vi "FuncVI_Sub - Script - Path argument to script path.vi"(6 "Allow Dialog (T)":bool=TRUE, 7 "CSE RefNum":T1, 8 "error in":errorcluster, 9 "prompt":string, 11 "arg: path":string) -> (0 "error out":errorcluster, 3 "script path":path)   [LabVIEW 2021]
doc: "::: CalcExpress Toolkit :::\nCopyright (c) 2000-2026 Konstantin Shifershteyn. All rights reserved."
uses:
  cse.llb/CSE Instance RefNum.ctl
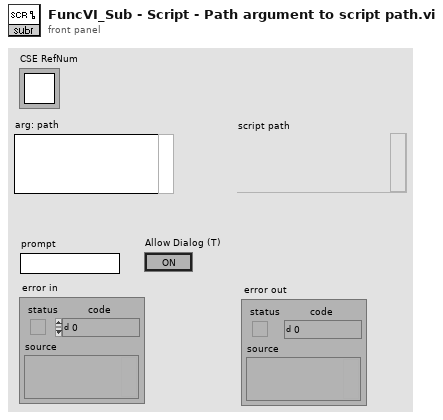
[diagram p1: front panel]
types:
  T1 = typedef "CSE Instance RefNum.ctl" = refnum<k1>
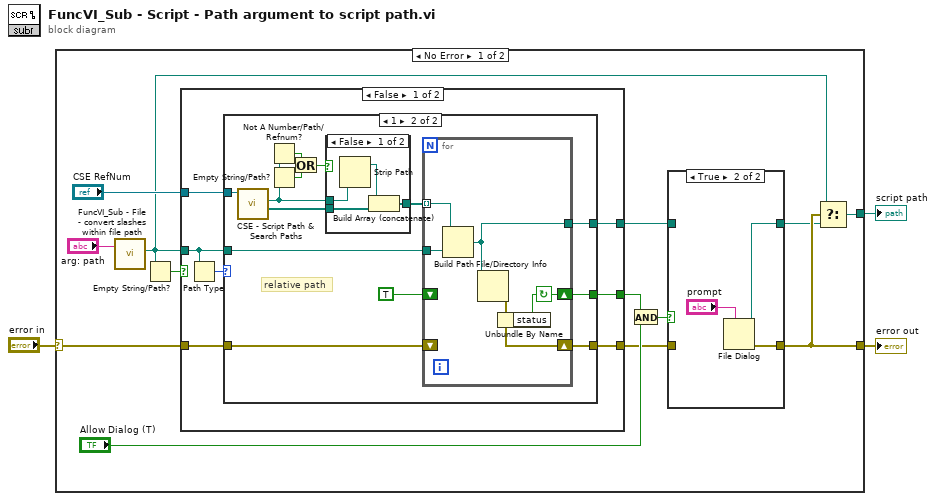
[diagram p0: block diagram]
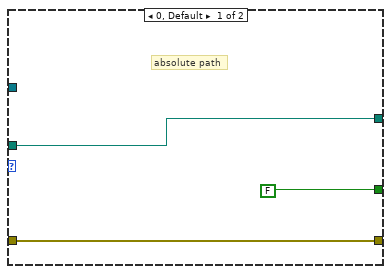
[diagram p3: hidden frame]
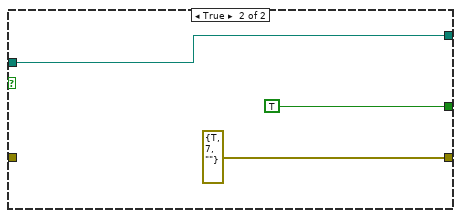
[diagram p5: hidden frame]
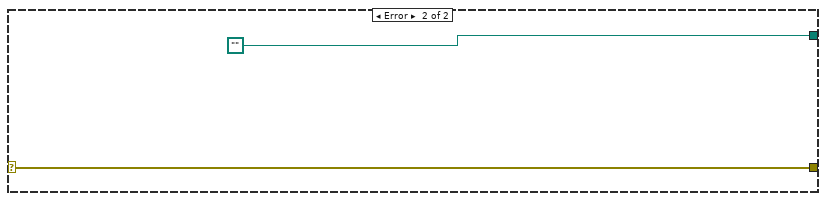
[diagram p6: hidden frame]
diagram:
  n1 = case shown="No Error" "error in" {
    selector: "error in" -> [w15 w58]
    tunnel: [w12 path ""] -> w3
    tunnel: [w6 w58] -> w2
    frame No Error {
      n2 = call "FuncVI_Sub - File - convert slashes within file path.vi"("str: path"="arg: path") -> ("path out"=w11:path)  [unwired: 3 in, 1 out]
      n3 = Empty String/Path?(string/path=w11) -> (empty?=w16:bool)
      n4 = case shown="False" w16 {
        tunnel: [w28 w55] -> w5
        tunnel: w11 -> [w23 w55]
        tunnel: w15 -> [w24 _]
        tunnel: [w25 errorcluster {"status"=TRUE, "code"=7, "source"=""} ("error out")] -> w7
        tunnel: "CSE RefNum" -> [w26 _]
        tunnel: [w22 TRUE] -> w10
        frame False {
          n5 = Path Type(1:w23) -> (0:w27:i16)
          n6 = case shown="1" w27 {
            tunnel: w23 -> [w30 w43]
            tunnel: [w30 w41] -> w28
            tunnel: w26 -> [_ w44]
            tunnel: [w31 w42] -> w25
            tunnel: w24 -> [w31 w33]
            tunnel: [FALSE w34] -> w22
            frame 0, Default {
              # "absolute path"
            }
            frame 1 {
              # "relative path"
              n7 = call "CSE - Script Path & Search Paths.vi"("CSE RefNum"=w44) -> ("search paths out"=w40:path[], "script file path out"=w37:path)  [unwired: 7 in, 2 out]
              n8 = Not A Number/Path/Refnum?(number/path/refnum=w37) -> (NaN/Path/Refnum?=w35:bool)
              n9 = Empty String/Path?(string/path=w37) -> (empty?=w36:bool)
              n10 = Or(x=w35, y=w36) -> (x .or. y?=w38:bool)
              n11 = case shown="False" w38 {
                tunnel: w40 -> [w53 w54]
                tunnel: [w52 w54] -> w39
                tunnel: w37 -> [w51 _]
                frame False {
                  n12 = Strip Path(path=w51) -> (stripped path=w50:path)  [unwired: 1 out]
                  n13 = Build Array (concatenate)(w50, w53) -> (w52:path[])
                }
                frame True {
                }
              }
              n14 = for {
                tunnel: w43 -> [w49]
                tunnel: w39 -> [w46] mode=indexing
                tunnel: [w47] -> w41
                shift-right: [w48] -> w42
                shift-left: w33 -> [_]
                shift-right: [w45] -> w34
                shift-left: TRUE -> [_]
                stop <- w45 continue-if-true
                n15 = Build Path(base path=w46, name or relative path=w49) -> (appended path=w47:path)
                n16 = File/Directory Info(path=w47) -> (error out=w48:errorcluster)  [unwired: 1 in, 6 out]
                n17 = Unbundle By Name(w48) -> ("status"=w45:bool)
              }
            }
          }
        }
        frame True {
        }
      }
      n18 = And(x=w10, y="Allow Dialog (T)") -> (x .and. y?=w8:bool)
      n19 = case shown="True" w8 {
        tunnel: w7 -> [w18 _]
        tunnel: [w18 w20] -> w6
        tunnel: w5 -> [w17 _]
        tunnel: [w17 w19] -> w4
        frame False {
        }
        frame True {
          n20 = File Dialog(7:"prompt") -> (0:w20:errorcluster, 3:w19:path)  [unwired: 6 in, 2 out]
        }
      }
      n21 = Select(t=w11, s=w6, f=w4) -> (s? t:f=w12:path)
    }
    frame Error {
    }
  }
  "script path" <- w3
  "error out" <- w2
